vi "Baseband Signal Generator.vi"(2 "Bit Rate(Rb)":dbl, 3 "Sampling Frequency(Fs)":dbl, 4 "Binary Input":i32[](array[numeric])) -> (0 "Baseband Signal":dbl[](array[numeric]), 1 "Samples per bit":i32)   [LabVIEW 2026]
panel:
  out "Baseband NRZ Signal":dbl[](graph)
  out "Total Samples":i32
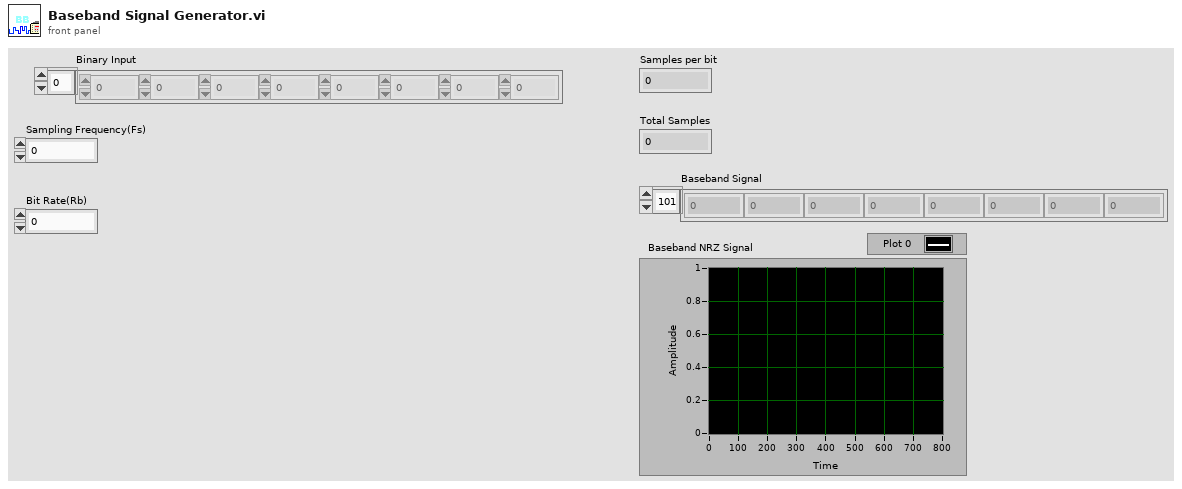
[diagram p1: front panel]
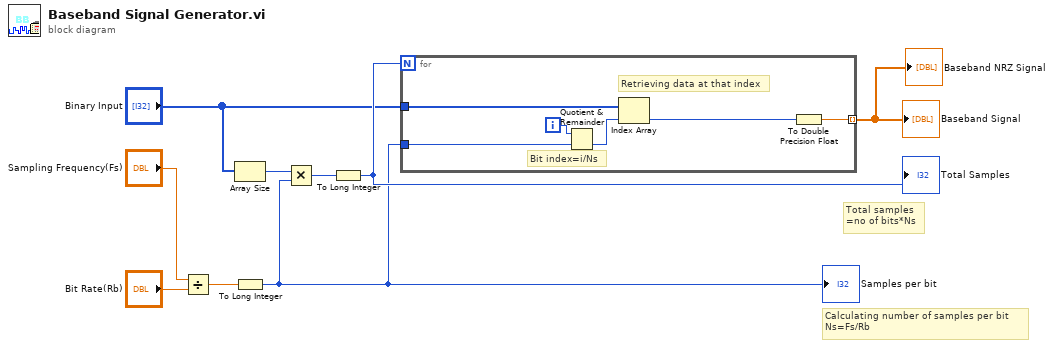
[diagram p0: block diagram]
diagram:
  # "Total samples\n=no of bits*Ns"
  # "Calculating number of samples per bit\nNs=Fs/Rb"
  n1 = Divide(x="Sampling Frequency(Fs)", y="Bit Rate(Rb)") -> (x/y=w7:dbl)
  n2 = Array Size(array="Binary Input") -> (size(s)=w6:i32)
  n3 = To Long Integer(number=w7) -> (32bit integer=w3:i32)
  "Samples per bit" <- w3
  n4 = Multiply(x=w6, y=w3) -> (x*y=w5:i32)
  n5 = To Long Integer(number=w5) -> (32bit integer=w4:i32)
  "Total Samples" <- w4
  n6 = for {
    N: w4 -> [_]
    tunnel: w3 -> [w14]
    tunnel: "Binary Input" -> [w13]
    tunnel: [w10] -> w1 mode=indexing
    i -> [w15]
    # "Retrieving data at that index"
    # "Bit index=i/Ns"
    n7 = Quotient & Remainder(x=w15, y=w14) -> (floor(x/y)=w12:i32)  [unwired: 1 out]
    n8 = Index Array(array=w13, index=w12) -> (element=w11:i32)
    n9 = To Double Precision Float(number=w11) -> (double precision float=w10:dbl)
  }
  "Baseband Signal" <- w1
  "Baseband NRZ Signal" <- w1
